vi "Encode Parameters into Words for Labels in a Channel.vi"(6 "modified indices":i32[](array[numeric]), 7 "reset index":bool, 8 "error in (no error)":errorcluster, 9 "labels settings for RT in":T1[](array[typedef]) {"Label Timestamp Channel Data Reference" format="%.0x"; "Word Initial Raw Value" format="%032.0f"; "Label Disable/Trigger Channel Reference" format="%.0x"; "parameter driver data"."Tx parameter refs" format="%.0x"; "SDI" format="%02b"; "label" format="%.0o"}, 11 "Parameter Values in":dbl[](array[numeric])) -> (0 "error out":errorcluster, 1 "labels settings for RT out":T1[](array[typedef]) {"Label Timestamp Channel Data Reference" format="%.0x"; "Word Initial Raw Value" format="%032.0f"; "Label Disable/Trigger Channel Reference" format="%.0x"; "parameter driver data"."Tx parameter refs" format="%.0x"; "SDI" format="%02b"; "label" format="%.0o"}, 2 "data words out":u32[](array[numeric]))   [LabVIEW 2020, in "AIM ARINC 429 Engine.lvlib" / "Implementation.lvlib" / "Tx Scheduled Labels Execution Unit.lvclass"]
uses:
  Tx Scheduled Labels Execution Unit.lvclass
  Shared/RT Label Settings.ctl
  Shared/Label.ctl
  Shared/RT Parameters.ctl
  Shared/Parameter Definition.ctl
  <vilib>/NI/NI VeriStand Encoding and Decoding/Encoding.ctl
  <vilib>/NI VeriStand/Custom Device API/Custom Device Item Ref.ctl
  Shared/Transfer Type.ctl
  <vilib>/NI VeriStand/Custom Device API/Data Reference.ctl
  Shared/Encode Parameter and Update Word (32-bit).vi/1445f95d-237d-4fc6-96b9-8992d347f513.vi
  Shared/Encode Parameter and Update Word (32-bit).vi/6b8853f0-8e5d-49e3-9391-4d3f8e5314b0.vi
  Shared/Encode Parameter and Update Word (32-bit).vi/2babc4f4-546e-4d35-846d-a4a1fbac0249.vi
  Shared/Encode Parameter and Update Word (32-bit).vi/1445f95d-237d-4fc6-96b9-8992d347f513.vi/9377bb8f-44b5-4a8f-87f1-966fd5a9edcc.vi
  Shared/Encode Parameter and Update Word (32-bit).vi/1445f95d-237d-4fc6-96b9-8992d347f513.vi/e95d9d1f-307c-44d6-9f26-c3f519a4990d.vi
  Shared/Encode Parameter and Update Word (32-bit).vi/1445f95d-237d-4fc6-96b9-8992d347f513.vi/0c23f515-4369-4514-bc3d-4444e6b437b2.vi
  Shared/Encode Parameter and Update Word (32-bit).vi/6b8853f0-8e5d-49e3-9391-4d3f8e5314b0.vi/136dcdcb-2dd3-4a4d-a796-a8f7a3f8e1ac.vi
  Shared/Encode Parameter and Update Word (32-bit).vi/6b8853f0-8e5d-49e3-9391-4d3f8e5314b0.vi/a54b505c-1216-4ef4-8378-3ceda9d188df.vi
  <vilib>/NI/NI VeriStand Encoding and Decoding/Get Bits Per Digit from Base.vi
  <vilib>/NI/NI VeriStand Encoding and Decoding/Encoding and Decoding.lvlib
  <vilib>/NI VeriStand/Custom Device API/Custom Device API.lvlib
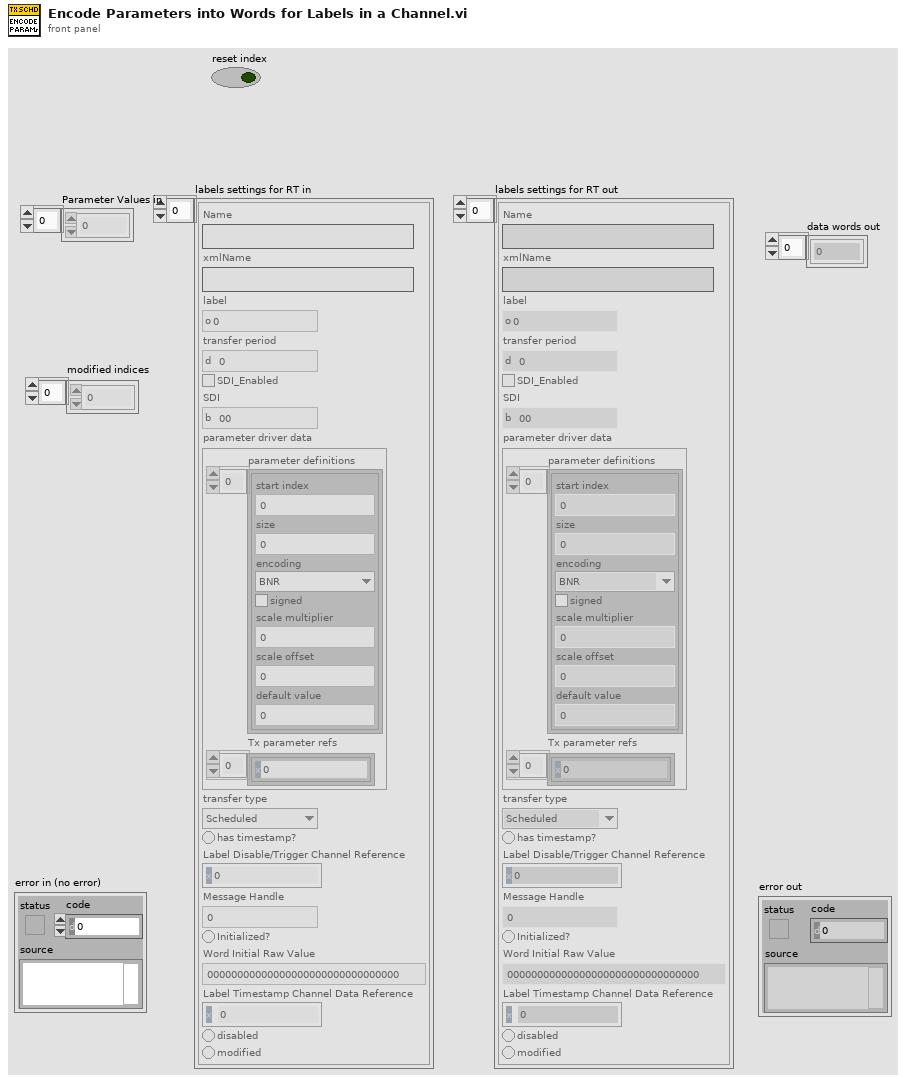
[diagram p1: front panel]
types:
  T1 = typedef "RT Label Settings.ctl" = cluster{"Name":string, "xmlName":string, "label":T2, "transfer period":u32, "SDI_Enabled":bool, "SDI":u8, "parameter driver data":T3, "transfer type":T7, "has timestamp?":bool, "Label Disable/Trigger Channel Reference":T6, "Message Handle":u64, "Initialized?":bool, "Word Initial Raw Value":u32, "Label Timestamp Channel Data Reference":T8, "disabled":bool, "modified":bool}
  T2 = typedef "Label.ctl" = u8
  T3 = typedef "RT Parameters.ctl" = cluster{"parameter definitions":T4[], "Tx parameter refs":T6[]}
  T4 = typedef "Parameter Definition.ctl" = cluster{"start index":i32, "size":i32, "encoding":T5, "signed":bool, "scale multiplier":dbl, "scale offset":dbl, "default value":dbl}
  T5 = typedef "Encoding and Decoding.lvlib/Encoding.ctl" = enum16{"BNR", "BCD", "Discrete"}
  T6 = typedef "Custom Device API.lvlib/Custom Device Item Ref.ctl" = u64
  T7 = typedef "Transfer Type.ctl" = enum16{"Scheduled", "Acyclic", "Block", "Strobe"}
  T8 = typedef "Custom Device API.lvlib/Data Reference.ctl" = i32
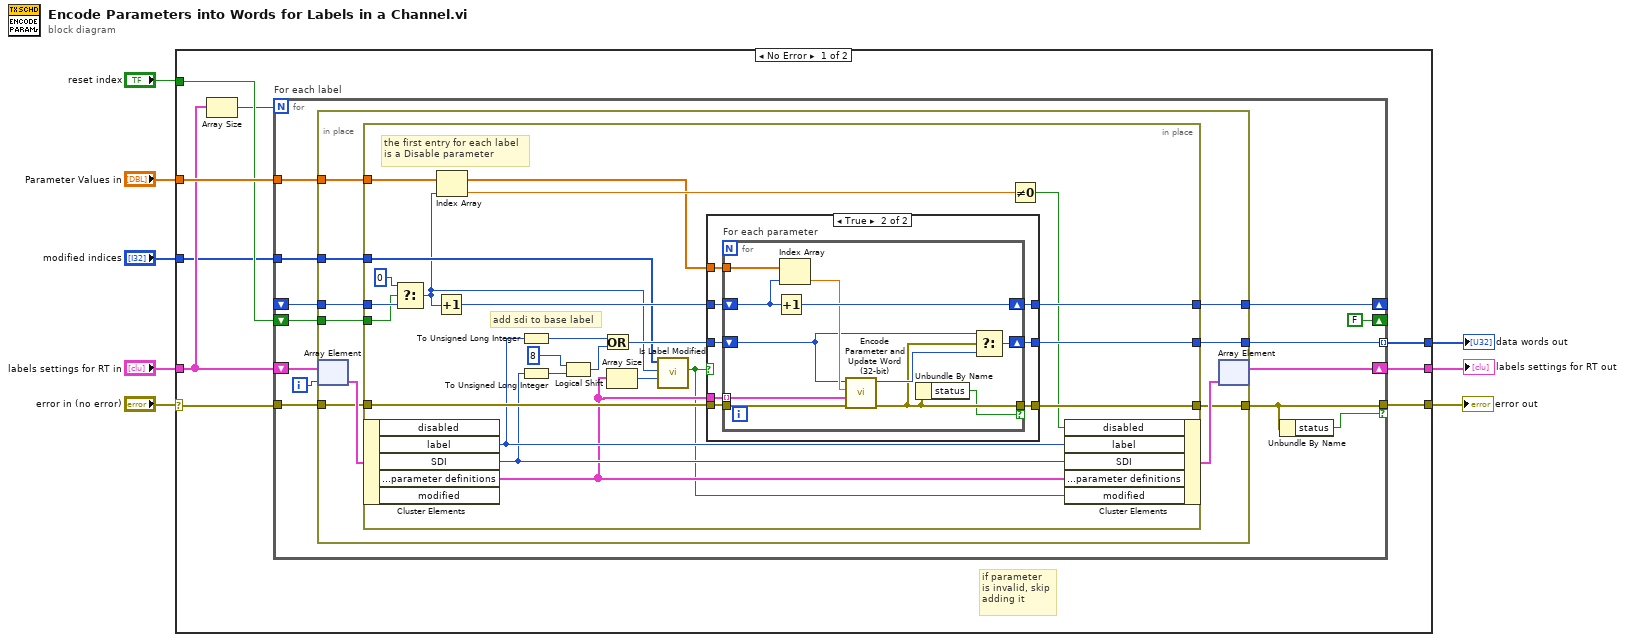
[diagram p0: block diagram]
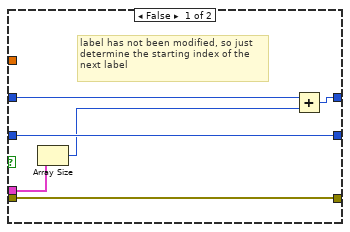
[diagram p2: hidden frame]
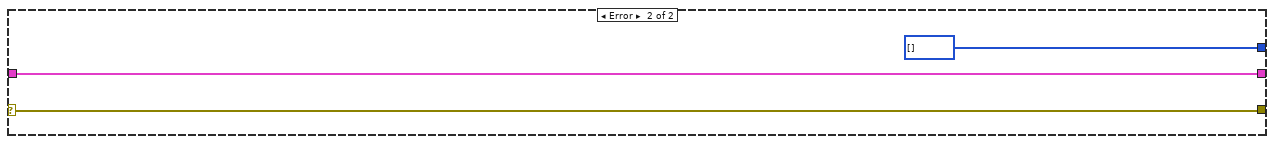
[diagram p3: hidden frame]
diagram:
  n1 = case shown="No Error" "error in (no error)" {
    selector: "error in (no error)" -> [w10 w91]
    tunnel: [w17 w91] -> w8
    tunnel: "Parameter Values in" -> [w16 _]
    tunnel: "reset index" -> [w15 _]
    tunnel: [w14 u32[] []] -> w5
    tunnel: [w13 w90] -> w4
    tunnel: "labels settings for RT in" -> [w11 w90]
    tunnel: "modified indices" -> [w9 _]
    frame No Error {
      # "if parameter\nis invalid, skip\nadding it"
      n2 = Array Size(array=w11) -> (size(s)=w12:i32)
      n3 = for "For each label" {
        N: w12 -> [_]
        shift-right: [FALSE ("reset index")] -> _
        shift-left: w15 -> [w24]
        tunnel: w16 -> [w28]
        shift-right: [w25] -> _
        shift-left: _ -> [w27]
        tunnel: [w22] -> w14 mode=indexing
        shift-right: [w21] -> w13
        shift-left: w11 -> [w30]
        tunnel: w10 -> [w26]
        tunnel: [w20] -> w17 if=w19
        tunnel: w9 -> [w18]
        i -> [w29]
        n4 = in-place {
          in-place-border: w28 -> [w38]
          in-place-border: w27 -> [w37]
          in-place-border: w26 -> [w36]
          in-place-border: [w35] -> w25
          in-place-border: w24 -> [w34]
          in-place-border: [w33] -> w22
          in-place-border: [w32] -> w20
          in-place-border: w18 -> [w31]
          n5 = in-place-array #1(w30, w29) -> (w40:T1)
          n6 = in-place {
            in-place-border: w38 -> [w60]
            in-place-border: w37 -> [w62]
            in-place-border: w36 -> [w59]
            in-place-border: [w58] -> w35
            in-place-border: w34 -> [w57]
            in-place-border: [w56] -> w33
            in-place-border: [w54] -> w32
            in-place-border: w31 -> [w43]
            # "add sdi to base label"
            # "the first entry for each label\nis a Disable parameter"
            n7 = in-place-cluster #2(w40) -> ("label"=w55:T2, "SDI"=w53:u8, "parameter driver data.parameter definitions"=w46:T4[])  [unwired: 2 out]
            n8 = Select(t=0 ("index"), s=w57, f=w62) -> (s? t:f=w42:i32)
            n9 = Increment(x=w42) -> (x+1=w47:i32)
            n10 = Index Array(array=w60, index=w42) -> (element=w61:dbl)
            n11 = To Unsigned Long Integer(number=w55) -> (unsigned 32bit integer=w50:u32)
            n12 = To Unsigned Long Integer(number=w53) -> (unsigned 32bit integer=w52:u32)
            n13 = Logical Shift(y=i16 8, x=w52) -> (x << y=w51:u32)
            n14 = Or(x=w50, y=w51) -> (x .or. y?=w49:u32)
            n15 = Array Size(array=w46) -> (size(s)=w41:i32)
            n16 = call "Is Label Modified.vi"("number of parameters"=w41, "initial index"=w42, "modified indices"=w43) -> ("label modified"=w44:bool)  [unwired: 8 in]
            n17 = case shown="True" w44 {
              tunnel: w60 -> [_ w77]
              tunnel: w59 -> [w67 w76]
              tunnel: [w65 w75] -> w58
              tunnel: [w66 w74] -> w56
              tunnel: [w67 w73] -> w54
              tunnel: w49 -> [w66 w72]
              tunnel: w47 -> [w68 w71]
              tunnel: w46 -> [w69 w70]
              frame False {
                # "label has not been modified, so just\ndetermine the starting index of the\nnext label"
                n18 = Array Size(array=w69) -> (size(s)=w64:i32)
                n19 = Add(x=w68, y=w64) -> (x+y=w65:i32)
              }
              frame True {
                n20 = for "For each parameter" {
                  shift-right: [w87] -> w75
                  shift-left: w71 -> [w78]
                  tunnel: w77 -> [w88]
                  tunnel: w70 -> [w85] mode=indexing
                  shift-right: [w81] -> w74
                  shift-left: w72 -> [w82]
                  tunnel: w76 -> [w84]
                  tunnel: [w80] -> w73 if=w79
                  n21 = Increment(x=w78) -> (x+1=w87:i32)
                  n22 = Index Array(array=w88, index=w78) -> (element=w86:dbl)
                  n23 = call "Encode Parameter and Update Word (32-bit).vi"("error in"=w84, "parameter definition"=w85, "parameter value"=w86, "word in"=w82) -> ("error out"=w80:errorcluster, "word out"=w83:u32)  [unwired: 6 in]
                  n24 = Unbundle By Name(w80) -> ("status"=w79:bool)
                  n25 = Select(t=w82, s=w80, f=w83) -> (s? t:f=w81:u32)
                }
              }
            }
            n26 = Not Equal To 0?(x=w61) -> (x != 0?=w45:bool)
            n27 = in-place-cluster #2("disabled"=w45, "label"=w55, "SDI"=w53, "parameter driver data.parameter definitions"=w46, "modified"=w44) -> (w39:T1)
          }
          n28 = in-place-array #1(w39) -> (w21:T1[])  [unwired: 1 out]
        }
        n29 = Unbundle By Name(w20) -> ("status"=w19:bool)
      }
    }
    frame Error {
    }
  }
  "data words out" <- w5
  "error out" <- w8
  "labels settings for RT out" <- w4
